vi "Module Init.vi"(8 "error in (no error)":errorcluster, 11 "Historian Charting Manager in":refnum<class "Historian Charting Manager.lvclass">) -> (0 "error out":errorcluster, 3 "Historian Charting Manager out":refnum<class "Historian Charting Manager.lvclass">)   [LabVIEW 2020, in "VolatusGUI.lvlib" / "Historian Charting Manager.lvclass"]
uses:
  Historian Charting Manager.lvclass
  C:/dev/lv20CE/relink/lv-volatus/Volatus/Module/Module.lvclass
  Volatus/Module/Module.lvclass/Module.ctl
  Volatus/MessageQ/MessageQ.lvclass/MessageQ.ctl
  Volatus/Module/Self Q.vi
  Volatus/MessageQ/Send.vi
  Historian Charting Manager.lvclass/Historian Charting Manager.ctl
  Volatus/Module/Module.lvclass
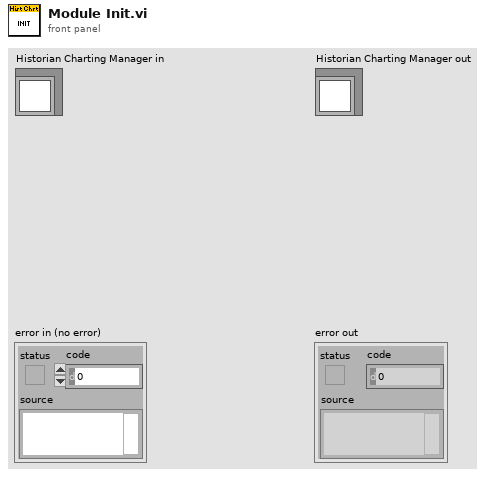
[diagram p1: front panel]
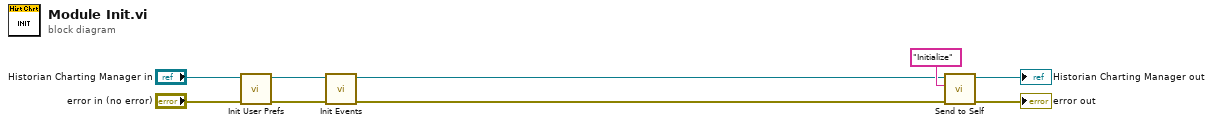
[diagram p0: block diagram]
diagram:
  n1 = call "Init User Prefs.vi"("error in (no error)"="error in (no error)", "Historian Charting Manager in"="Historian Charting Manager in") -> ("error out"=w3:errorcluster, "Historian Charting Manager out"=w1:refnum<class "Historian Charting Manager.lvclass">)  [unwired: 8 in]
  n2 = call "Init Events.vi"("error in (no error)"=w3, "Historian Charting Manager in"=w1) -> ("error out"=w5:errorcluster, "Historian Charting Manager out"=w4:refnum<class "Historian Charting Manager.lvclass">)  [unwired: 8 in]
  n3 = call "Send to Self.vi"("error in (no error)"=w5, "Message ID"="Initialize", "Module in"=w4) -> ("error out"=→"error out":errorcluster, "Module out"=→"Historian Charting Manager out":refnum<class "Historian Charting Manager.lvclass">)  [unwired: 7 in]
